vi "to string 3.1.vi"(8 "error in":errorcluster, 10 "data in":string, 11 "Shared Memory configuration in":refnum<class "Shared Memory configuration.lvclass">) -> (0 "error out":errorcluster, 2 "data out":string, 3 "Shared Memory configuration out":refnum<class "Shared Memory configuration.lvclass">)   [LabVIEW 2014, in "Shared Memory configuration.lvclass"]
uses:
  Shared Memory configuration.lvclass
  Shared Memory configuration.lvclass/Shared Memory configuration.ctl
  <vilib>/NI/Configuration Framework/serializable configuration/NISE_CEF_serializable configuration.lvclass
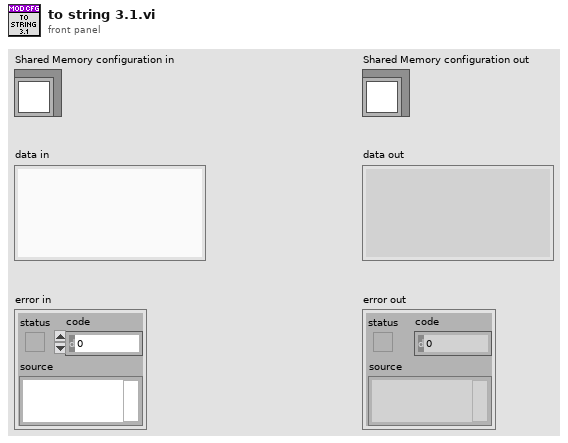
[diagram p1: front panel]
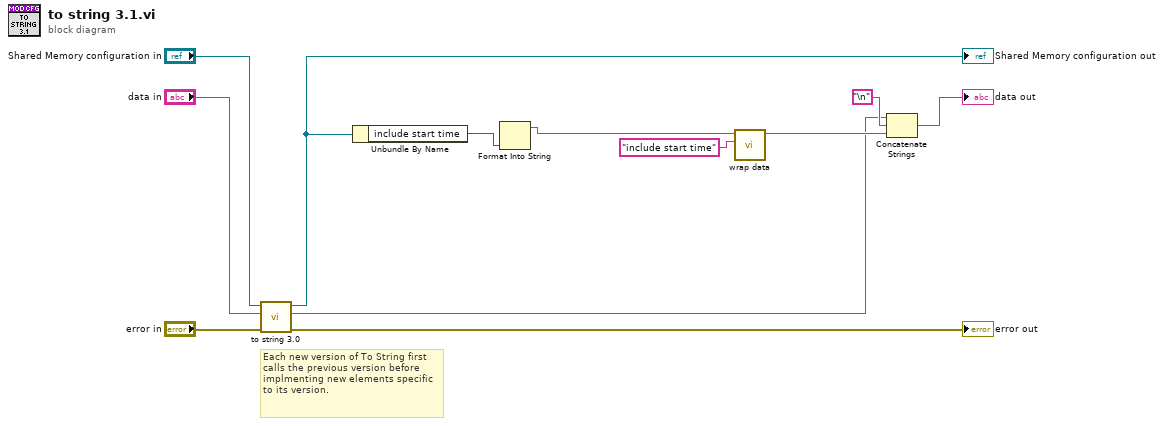
[diagram p0: block diagram]
diagram:
  # "Each new version of To String first calls the previous version before implmenting new elements specific to its version."
  n1 = call "to string 3.0.vi"("error in"="error in", "data in"="data in", "Shared Memory configuration in"="Shared Memory configuration in") -> ("error out"=→"error out":errorcluster, "data out"=w3:string, "Shared Memory configuration out"=w6:refnum<class "Shared Memory configuration.lvclass">)  [unwired: 6 in]
  "Shared Memory configuration out" <- w6
  n2 = Unbundle By Name(w6) -> ("include start time"=w2:bool)
  n3 = Format Into String(w2) -> (resulting string=w1:string)  [unwired: 3 in, 1 out]
  n4 = call <vilib>:"wrap data.vi"("identifier"="include start time", "data to wrap"=w1) -> ("wrapped data"=w9:string)  [unwired: 9 in]
  n5 = Concatenate Strings(w3, "\n", w9) -> (→"data out":string)
